vi "Connect.vi"(8 "error in (no error)":errorcluster, 11 "object in":refnum<class "AIO_Channel.lvclass">) -> (0 "error out":errorcluster, 2 "Success?":bool, 3 "object out":refnum<class "AIO_Channel.lvclass">)   [LabVIEW 2021, in "DAQmx.lvlib" / "AIO_Channel.lvclass"]
uses:
  AIO_Channel.lvclass
  AIO_Channel.lvclass/AIO_Channel.ctl
  AIO-Configuration_class/AIO-Configuration.lvclass
  C:/Users/averna/Documents/LV Gym DEMO/Factory Pattern/Device Channels/Dependencies/AIO-Channel.lvlibp/Channels/AIO-Channel/AIO-Configuration_class/AIO-Configuration.lvclass
  Properties/Get-AIO-DAQmx-Cfg.vi
  <vilib>/DAQmx/create/channels.llb/DAQmx Create Channel (AI-Voltage-Basic).vi
  <vilib>/DAQmx/create/channels.llb/DAQmx Create Channel (AO-Voltage-Basic).vi
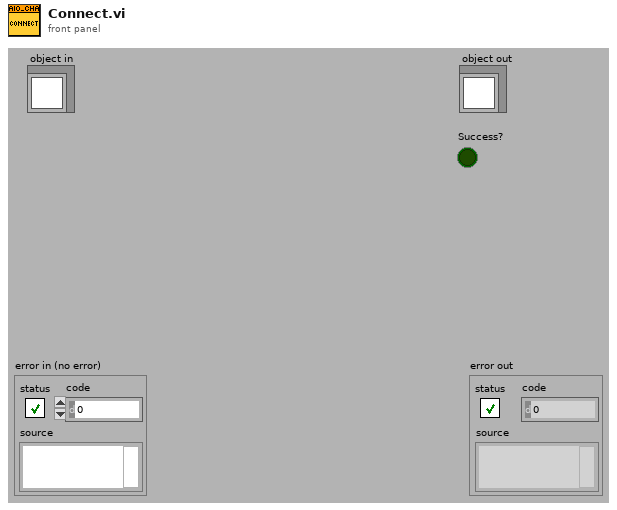
[diagram p1: front panel]
types:
  T1 = typedef "AIO-Channel.lvlibp/AIO-Configuration.lvclass/Direction.ctl" = enum16{"Input", "Output"}
  T2 = typedef "DAQmx.lvlib/AIO-Configuration.lvclass/Data.ctl" = cluster{"DAQ_Line":string, "maximum value":dbl, "minimum value":dbl, "input terminal configuration":i32, "custom scale name":string}
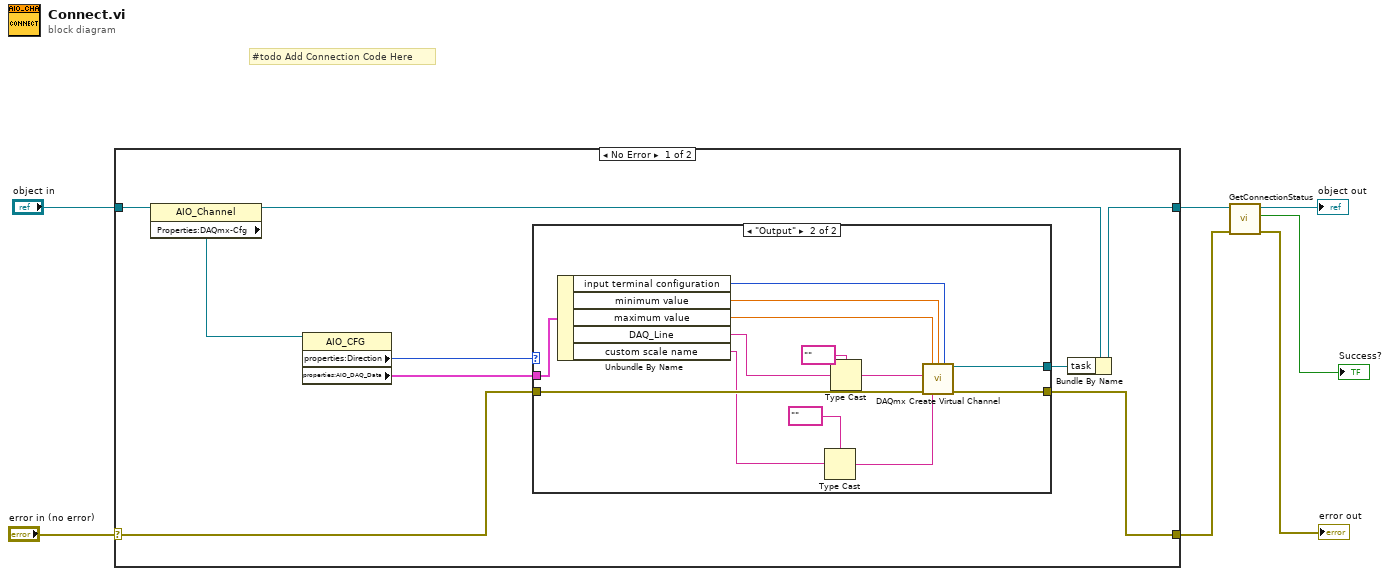
[diagram p0: block diagram]
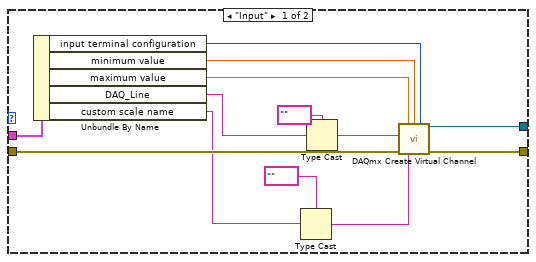
[diagram p2: hidden frame]
diagram:
  # "#todo Add Connection Code Here"
  n1 = case shown="No Error" "error in (no error)" {
    selector: "error in (no error)" -> [w9 w44]
    tunnel: [w10 w44] -> w3
    tunnel: [w15 w43] -> w5
    tunnel: "object in" -> [w16 w43]
    frame No Error {
      n2 = property class="AIO_Channel"(reference=w16) -> (reference out=w14:refnum<class "AIO_Channel.lvclass">, "Properties:DAQmx-Cfg"=w13:refnum<class "AIO-Configuration.lvclass">)  [unwired: 1 in, 1 out]
      n3 = property class="AIO_CFG"(reference=w13) -> ("properties:Direction"=w12:T1, "properties:AIO_DAQ_Data"=w8:T2)  [unwired: 1 in, 2 out]
      n4 = case shown="\"Output\"" w12 {
        tunnel: [w29 w42] -> w11
        tunnel: [w28 w41] -> w10
        tunnel: w9 -> [w27 w40]
        tunnel: w8 -> [w24 w37]
        frame "Input" {
          n5 = Unbundle By Name(w24) -> ("input terminal configuration"=w22:i32, "minimum value"=w21:dbl, "maximum value"=w20:dbl, "DAQ_Line"=w23:string, "custom scale name"=w17:string)
          n6 = Type Cast(type=tag "" ("custom scale name"), x=w17) -> (*(type *) &x=w19:tag)
          n7 = Type Cast(type=tag "" ("lines"), x=w23) -> (*(type *) &x=w25:tag)
          n8 = call-poly <vilib>:"DAQmx Create Virtual Channel.vi"("maximum value"=w20, "minimum value"=w21, "input terminal configuration"=w22, "physical channels"=w25, "error in"=w27, "custom scale name"=w19) -> ("task out"=w29:refnum<k21>, "error out"=w28:errorcluster)  [unwired: 8 in]
        }
        frame "Output" {
          n9 = Unbundle By Name(w37) -> ("input terminal configuration"=w35:i32, "minimum value"=w34:dbl, "maximum value"=w33:dbl, "DAQ_Line"=w36:string, "custom scale name"=w30:string)
          n10 = Type Cast(type=tag "" ("custom scale name"), x=w30) -> (*(type *) &x=w32:tag)
          n11 = Type Cast(type=tag "" ("lines"), x=w36) -> (*(type *) &x=w38:tag)
          n12 = call-poly <vilib>:"DAQmx Create Virtual Channel.vi"("maximum value"=w33, "minimum value"=w34, "output terminal configuration"=w35, "physical channels"=w38, "error in"=w40, "custom scale name"=w32) -> ("task out"=w42:refnum<k21>, "error out"=w41:errorcluster)  [unwired: 8 in]
        }
      }
      n13 = Bundle By Name(cluster=w14, "task"=w11) -> (w15:refnum<class "AIO_Channel.lvclass">)
    }
    frame Error {
    }
  }
  n14 = call-dynamic "GetConnectionStatus.vi"("error in (no error)"=w3, "object in"=w5) -> ("error out"=→"error out":errorcluster, "Connected?"=→"Success?":bool, "object out"=→"object out":refnum<class "AIO_Channel.lvclass">)  [unwired: 7 in]
